vi "Test_Bench_Pi.vi"() -> ()   [LabVIEW 2024]
panel:
  out "Array":string[][](array[string])
  in  "format string":string="%f"
  in  "file (use dialog)":path=path "C:/Users/Tanner/Desktop/Angelo/NMR/Variable Pi/Test.txt"
  out "output array":string[][](array[string])
  out "Numeric 2":i32
  in  "how many iterations":i32
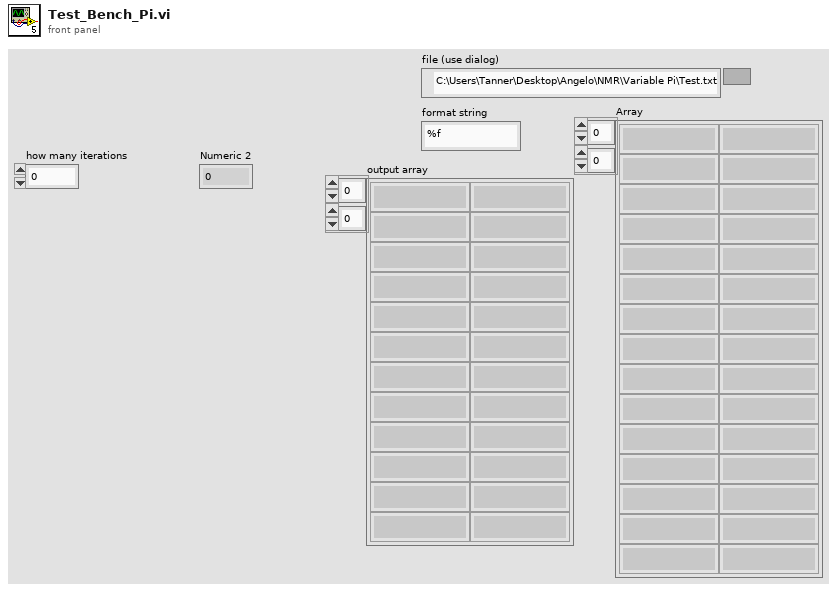
[diagram p1: front panel]
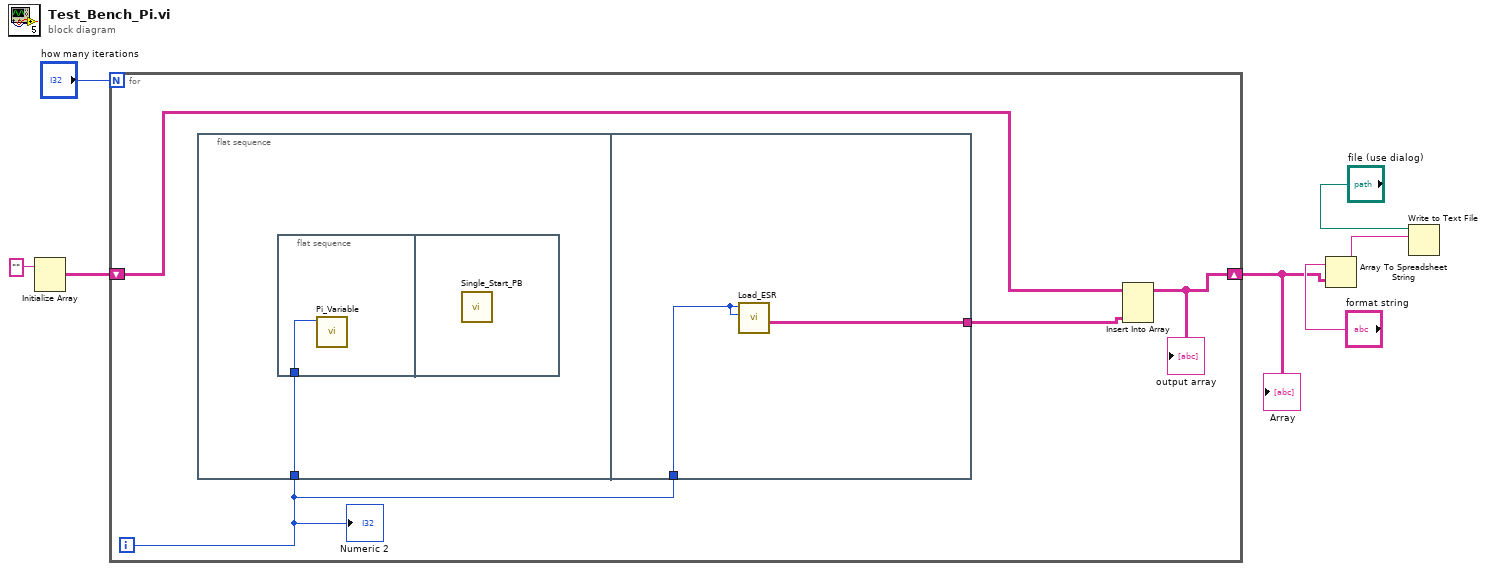
[diagram p0: block diagram]
diagram:
  n1 = Initialize Array("") -> (w5:string[][])  [unwired: 2 in]
  n2 = for {
    N: "how many iterations" -> [_]
    shift-right: [w8] -> w1
    shift-left: w5 -> [w10]
    i -> [w11]
    n3 = flat-sequence {
      tunnel: w11 -> [w12]
      tunnel: w11 -> [w15]
      tunnel: [w14] -> w9
      frame #0 {
        n4 = flat-sequence {
          tunnel: w12 -> [w13]
          frame #0 {
            n5 = call "Pi_Variable.vi"("Numeric"=w13) -> ()  [unwired: 11 in]
          }
          frame #1 {
            n6 = call "Single_Start_PB.vi"() -> ()  [unwired: 12 in]
          }
        }
      }
      frame #1 {
        n7 = call "Load_ESR.vi"("wait time adjustment (inverted)"=w15, "wait time adjustment"=w15) -> ("Array"=w14:string[][])  [unwired: 7 in, 2 out]
      }
    }
    n8 = Insert Into Array(array=w10, new element=w9) -> (w8:string[][])  [unwired: 2 in]
    "output array" <- w8
    "Numeric 2" <- w11
  }
  "Array" <- w1
  n9 = Array To Spreadsheet String(array=w1, 3:"format string") -> (spreadsheet string=w3:string)  [unwired: 1 in]
  n10 = Write to Text File(file (use dialog)="file (use dialog)", text=w3) -> ()  [unwired: 2 in, 3 out]
